vi "frw_csv_ini.vi"(8 "error in":errorcluster, 9 "eeg_device":T1, 10 "file_name":string, 11 "folder":path) -> (0 "error out":errorcluster, 3 "path out":path)   [LabVIEW 2013]
uses:
  gui/type_def/device.ctl
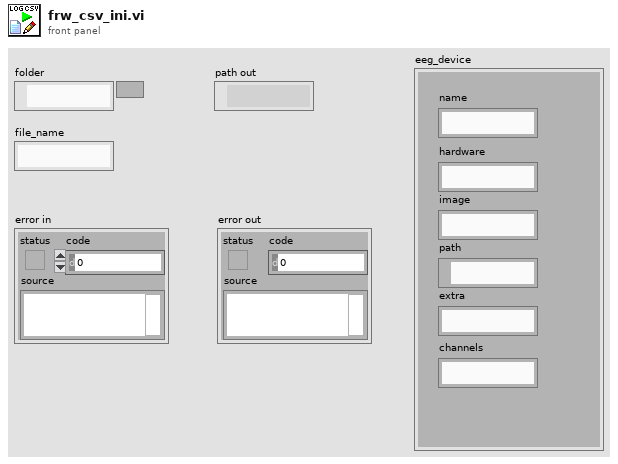
[diagram p1: front panel]
types:
  T1 = typedef "device.ctl" = cluster{"name":string, "hardware":string, "image":string, "path":path, "extra":string, "channels":string}
  T2 = enum16{"open", "replace", "create", "open or create", "replace or create", "replace or create with confirmation"}
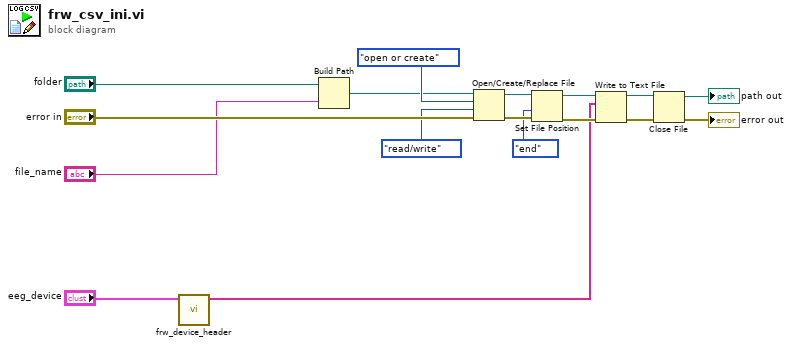
[diagram p0: block diagram]
diagram:
  n1 = call "frw_device_header.vi"("eeg_device"="eeg_device") -> ("header array"=w1:string[])  [unwired: 10 in]
  n2 = Build Path(base path="folder", name or relative path="file_name") -> (appended path=w4:path)
  n3 = Open/Create/Replace File(file path (use dialog)=w4, error in="error in", operation (0:open)=T2."open or create", access (0:read/write)=enum16{"read/write", "read-only", "write-only"}."read/write") -> (refnum out=w13:refnum<file>, error out=w15:errorcluster)  [unwired: 3 out]
  n4 = Set File Position(refnum=w13, from (0:start)=enum16{"start", "end", "current"}."end", error in=w15) -> (refnum out=w12:refnum<file>, error out=w11:errorcluster)  [unwired: 1 in]
  n5 = Write to Text File(file (use dialog)=w12, text=w1, error in=w11) -> (refnum out=w9:refnum<file>, error out=w10:errorcluster)  [unwired: 2 out]
  n6 = Close File(refnum=w9, error in=w10) -> (path=→"path out":path, error out=→"error out":errorcluster)
